vi "Payload to Real.vi"(3 "Payload":string) -> (1 "Real":dbl[](array[numeric]))   [LabVIEW 2019]
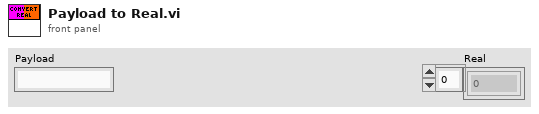
[diagram p1: front panel]
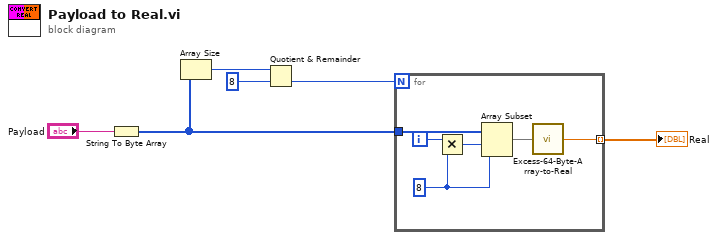
[diagram p0: block diagram]
diagram:
  n1 = String To Byte Array(string="Payload") -> (unsigned byte array=w6:u8[])
  n2 = Array Size(array=w6) -> (size(s)=w3:i32)
  n3 = Quotient & Remainder(x=w3, y=8) -> (floor(x/y)=w1:i32)  [unwired: 1 out]
  n4 = for {
    N: w1 -> [_]
    tunnel: w6 -> [w9]
    tunnel: [w8] -> w4 mode=indexing
    i -> [w12]
    w7 = 8 ("y")
    n5 = Multiply(x=w12, y=w7) -> (x*y=w10:i32)
    n6 = Array Subset(array=w9, index=w10, length=w7) -> (w11:u8[])
    n7 = call "Excess-64-Byte-Array-to-Real.vi"("Byte array (4 or 8 bytes)"=w11) -> ("Real Number"=w8:dbl)  [unwired: 4 in]
  }
  "Real" <- w4
